vi "Sub.vi"(7 "Gain":dbl, 11 "error in":errorcluster) -> (4 "Sum":dbl, 6 "Status":bool, 15 "error out":errorcluster)   [LabVIEW 2026]
doc: "Issue 136 subVI example, version 3: X removed, Sum is Gain plus one."
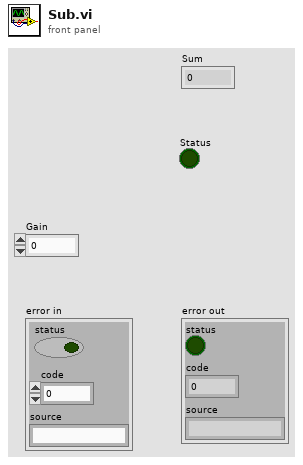
[diagram p1: front panel]
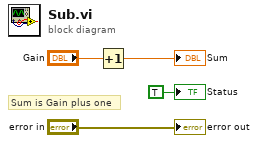
[diagram p0: block diagram]
diagram:
  # "Sum is Gain plus one"
  n1 = Increment(x="Gain") -> (x+1=→"Sum":dbl)
  "Status" <- TRUE ("ok")
  "error out" <- "error in"
